vi "Main (1553).vi"() -> ()   [LabVIEW 2020]
doc: "Use this template to build a simple state machine design pattern. Each state executes code and determines which state to transition to."
uses:
  1553/_controls/1553_formatting.ctl
  1553/_controls/1553_State.ctl
  1553/_controls/1553_Data.ctl
  1553/_controls/aim1553_cluster.ctl
  1553/_controls/aim1553_messages.ctl
  1553/_controls/1553_Parameters_key.ctl
  1553/_controls/1553_Parameters.ctl
  1553/_controls/1553_minorFrames.ctl
  1553/_controls/aim1553_RT_list.ctl
  1553/_controls/ballard1553_hw_map.ctl
  1553/_controls/ballard1553_RT_list.ctl
  1553/_controls/ballard1553_cluster.ctl
  <vilib>/Utility/error.llb/DialogType.ctl
  Libraries/Aim_1553_Parameter_ni/AIM_1553_Parameter_ni.lvlib
  Libraries/Ballard_1553_Parameter_ni/Ballard_1553_Parameter_ni.lvlib
  Libraries/Ballard_1553_Hardware_ni/Ballard_1553_Hardware_ni.lvlib
  <userlib>/_OpenG.lib/array/array.llb/Sort 1D Array (DBL)__ogtk.vi
  <userlib>/_OpenG.lib/array/array.llb/Remove Duplicates from 1D Array (Variant)__ogtk.vi
  <userlib>/_OpenG.lib/array/array.llb/Search 1D Array (DBL)__ogtk.vi
  <userlib>/_OpenG.lib/array/array.llb/Index 1D Array Elements (DBL)__ogtk.vi
panel:
  out "db read time mS":u32
  in  "formatting":T1=enum."ni-AIM"
  in  "Configure SelfTestBus?":bool
  out "Progress":string
  in  "Stop Button":bool
  in  "Generate XMLs":bool
  in  "Source Filepath (xlsx)":path=path "C:/Users/Administrator/Desktop/GIT/1553-Configurator/docs/example configurations/_template_Ballard_1553.xlsx"
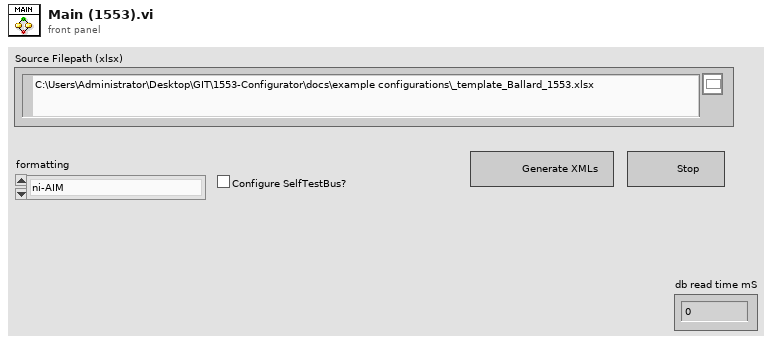
[diagram p1: front panel]
types:
  T1 = typedef "1553_formatting.ctl" = enum16{"ni-Ballard", "ni-AIM"}
  T2 = typedef "DialogType.ctl" = u16
  T3 = typedef "1553_Data.ctl" = cluster{"Database Filepath (xlsx)":path, "formatting":T1, "parameter config - aim":T4[], "hw config - aim":T9[], "hw config - ballard":T10[], "parameter config - ballard":T12[]}
  T4 = typedef "aim1553_cluster.ctl" = cluster{"messages":map{string, T5}, "parameters":map{T6, T7[]}, "frames":map{string, map{string, T8}}}
  T5 = typedef "aim1553_messages.ctl" = cluster{"messageType":string, "TA1":i32, "SA1":i32, "words":i32, "TA2":i32, "SA2":i32, "MC":i32, "direction":string}
  T6 = typedef "1553_Parameters_key.ctl" = cluster{"TA":i32, "SA":i32}
  T7 = typedef "1553_Parameters.ctl" = cluster{"name":string, "encoding":string, "signed":bool, "startBit":i32, "numberOfBits":i32, "scale":dbl, "offset":dbl, "unit":string, "defaultValue":dbl}
  T8 = typedef "1553_minorFrames.ctl" = cluster{"MessageNames":string[], "FramePeriodUs":i32}
  T9 = typedef "aim1553_RT_list.ctl" = cluster{"terminalAddress":i32[]}
  T10 = typedef "ballard1553_hw_map.ctl" = map{i32, T11}
  T11 = typedef "ballard1553_RT_list.ctl" = cluster{"terminalAddress":i32[], "channel":i32}
  T12 = typedef "ballard1553_cluster.ctl" = cluster{"messages":map{string, T5}, "parameters":map{T6, T7[]}, "frames":map{string, map{string, T8}}}
  T13 = typedef "1553_State.ctl" = enum16{"Initialize", "Wait for Event", "Read Source Files", "Validate Data", "Write Configuration Files", "Exit"}
  T14 = enum8{"Enabled", "Disabled", "Disabled and Grayed Out"}
  T15 = enum32{"invalid app kind", "Development System", "Run Time System", "Student Edition", "Embedded LabVIEW", "Evaluation", "Custom"}
  T16 = typedef "Database_Array.ctl" = cluster{"Core Number":i32, "Channel Number":i32, "Channel Name":string, "Channel Speed":i32, "Label Decimal":i32, "Label Name":string, "Min Rate (mS)":i32, "Max Rate (mS)":i32, "SDI":i32, "SSM":i32, "Create SDI":bool, "Create SSM":bool, "Create Parity":bool, "Parameter Name":string, "Start Bit":i32, "Number of Bits":i32, "Scale":string, "Offset":string, "Signed":bool, "Unit":string, "Encoding":T17, "Default Value":string}
  T17 = typedef "Encoding.ctl" = enum16{"BCD", "BNR", "Discrete"}
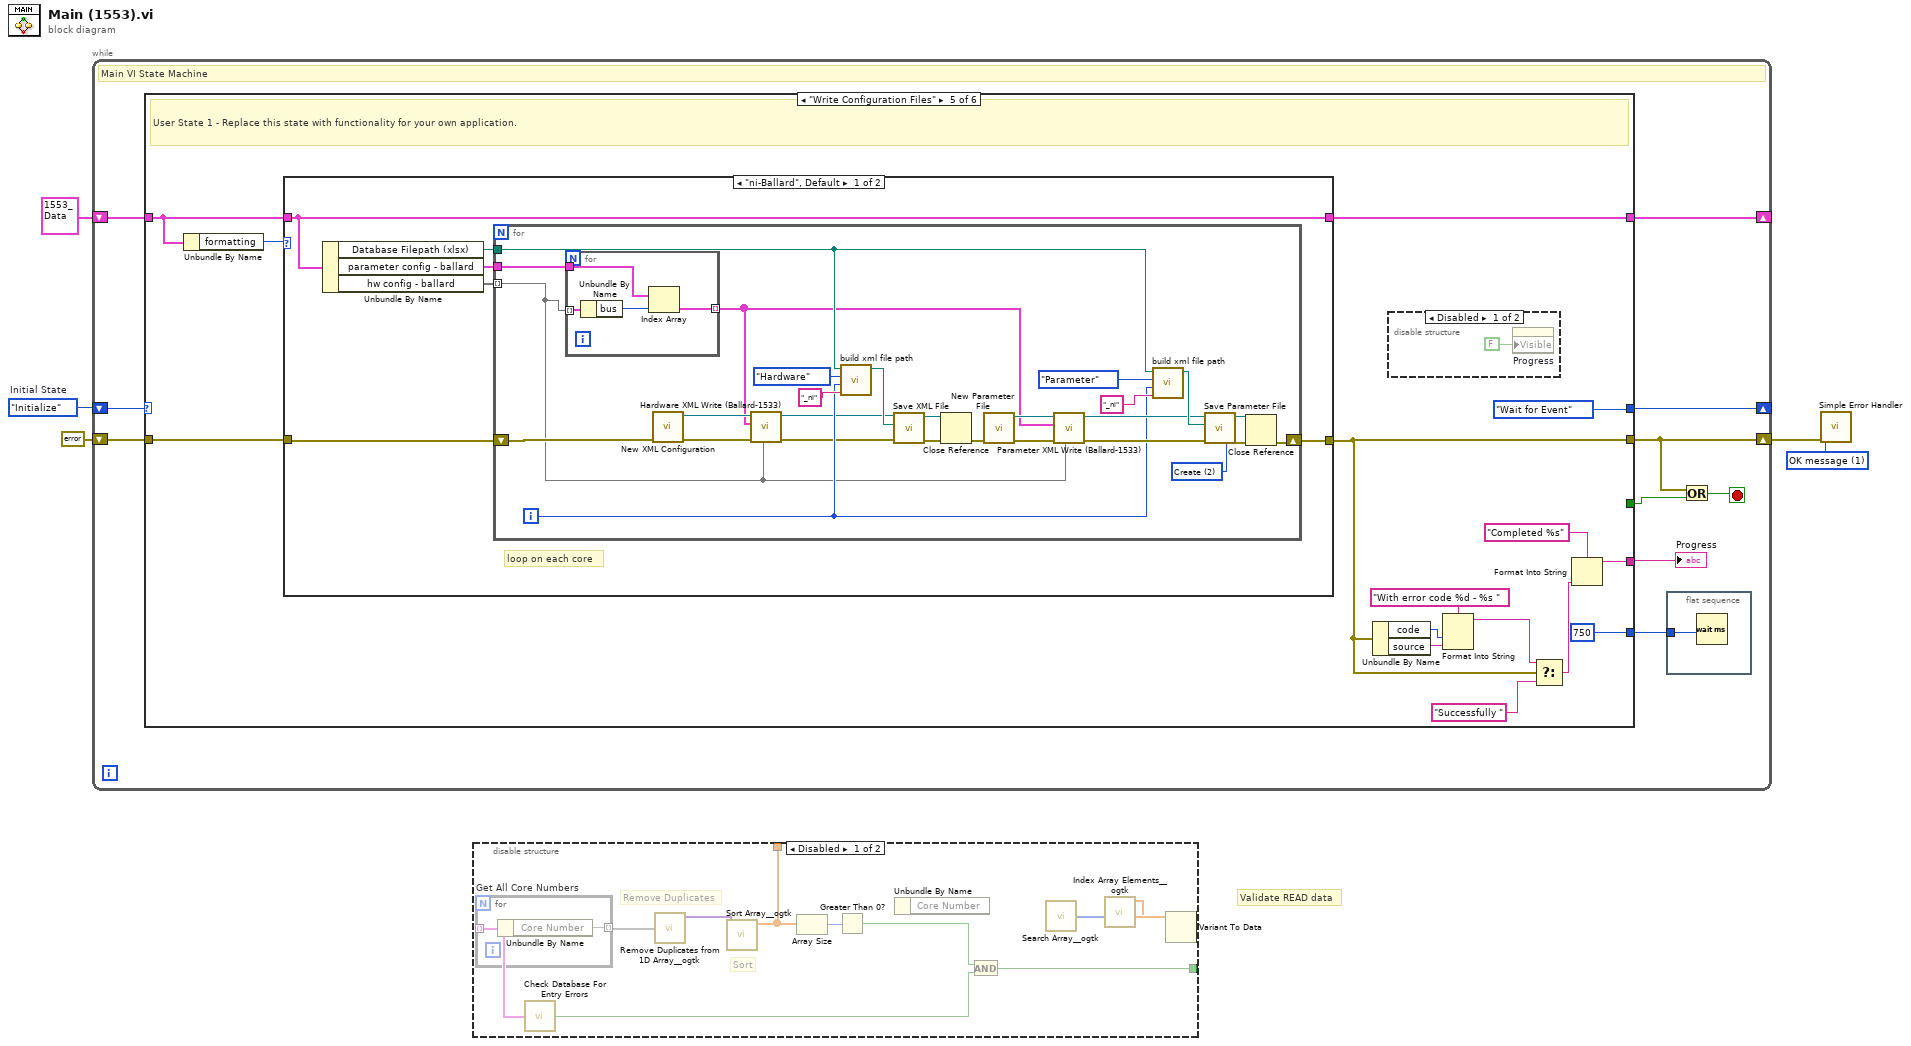
[diagram p0: block diagram]
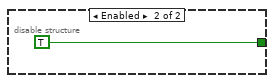
[diagram p2: hidden frame]
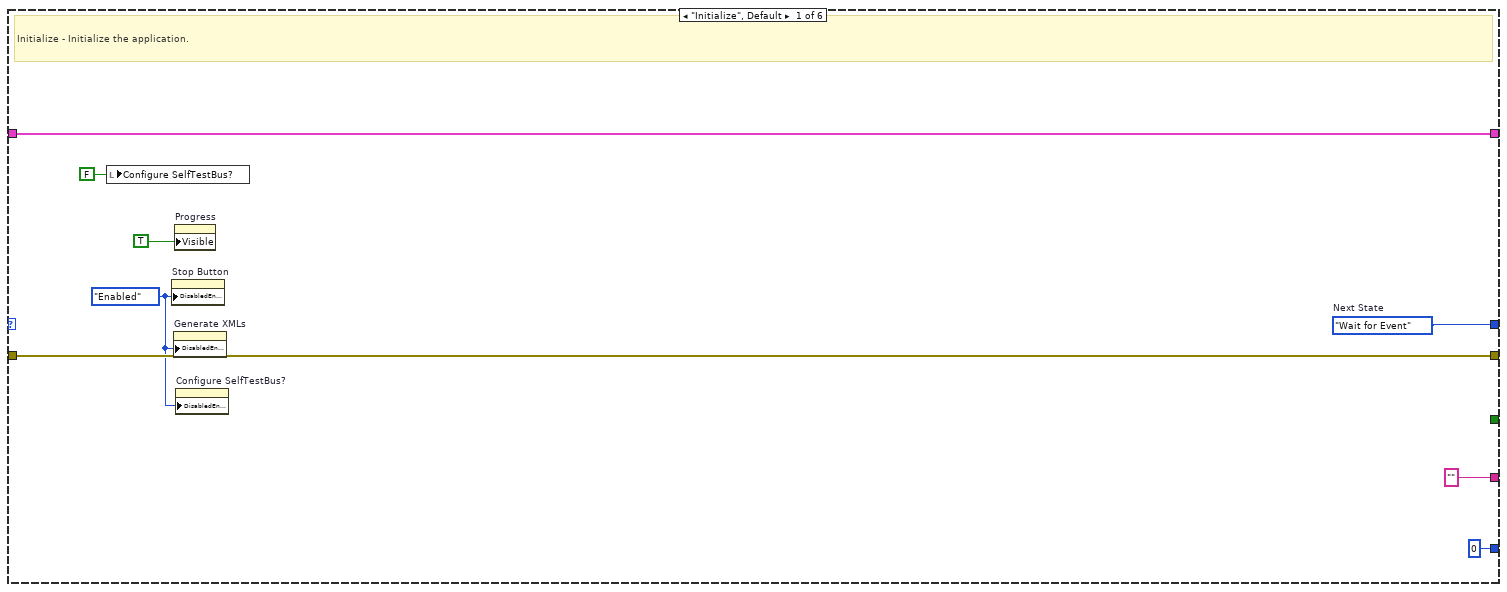
[diagram p3: hidden frame]
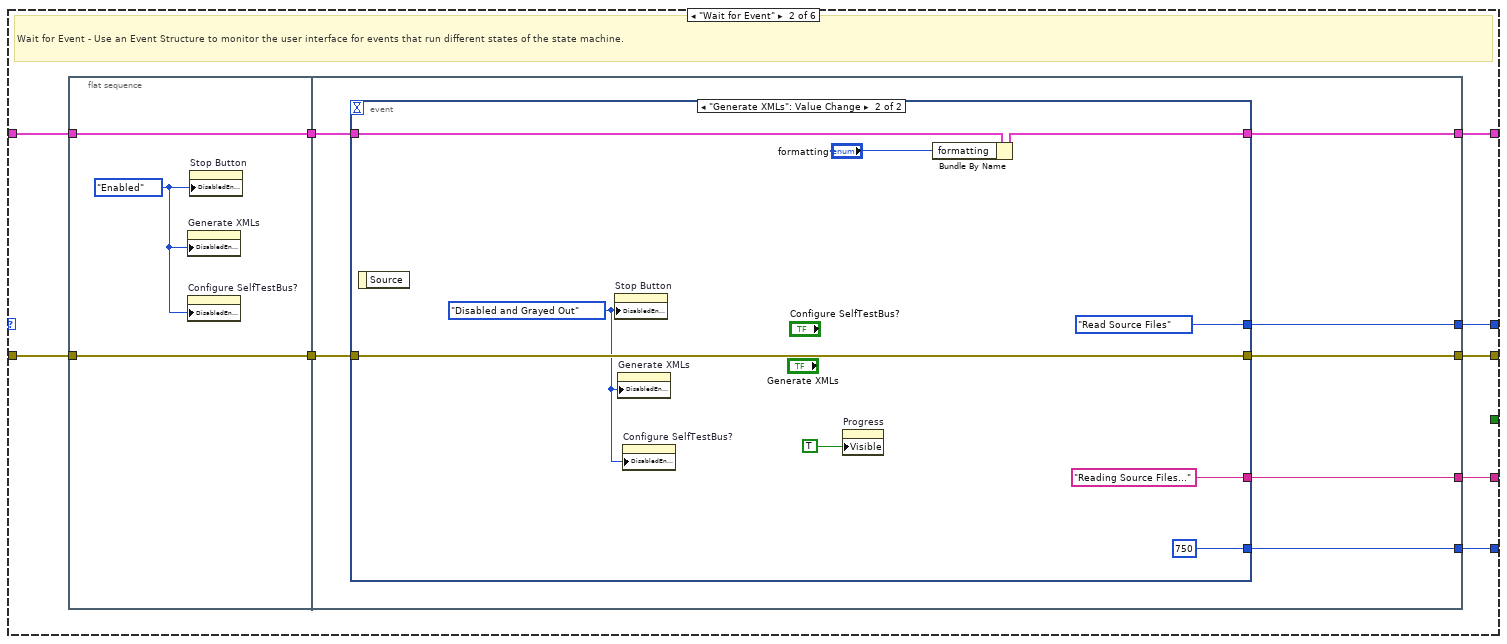
[diagram p4: hidden frame]
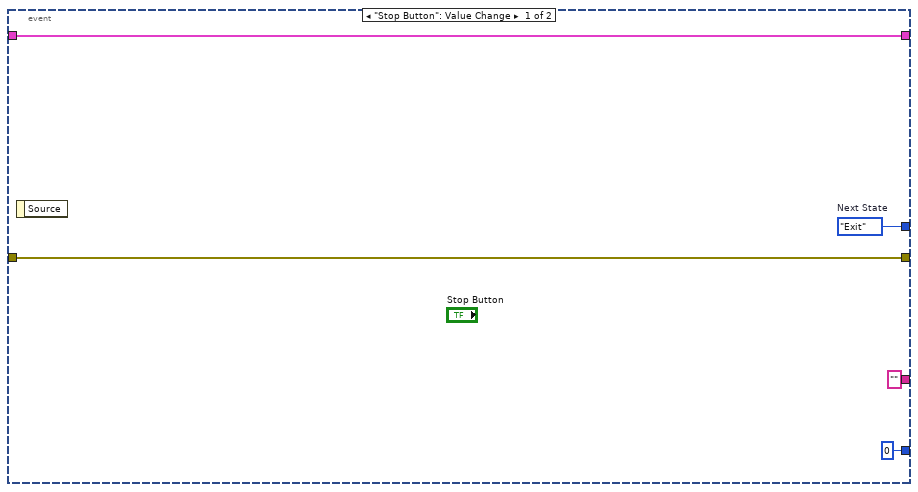
[diagram p5: hidden frame]
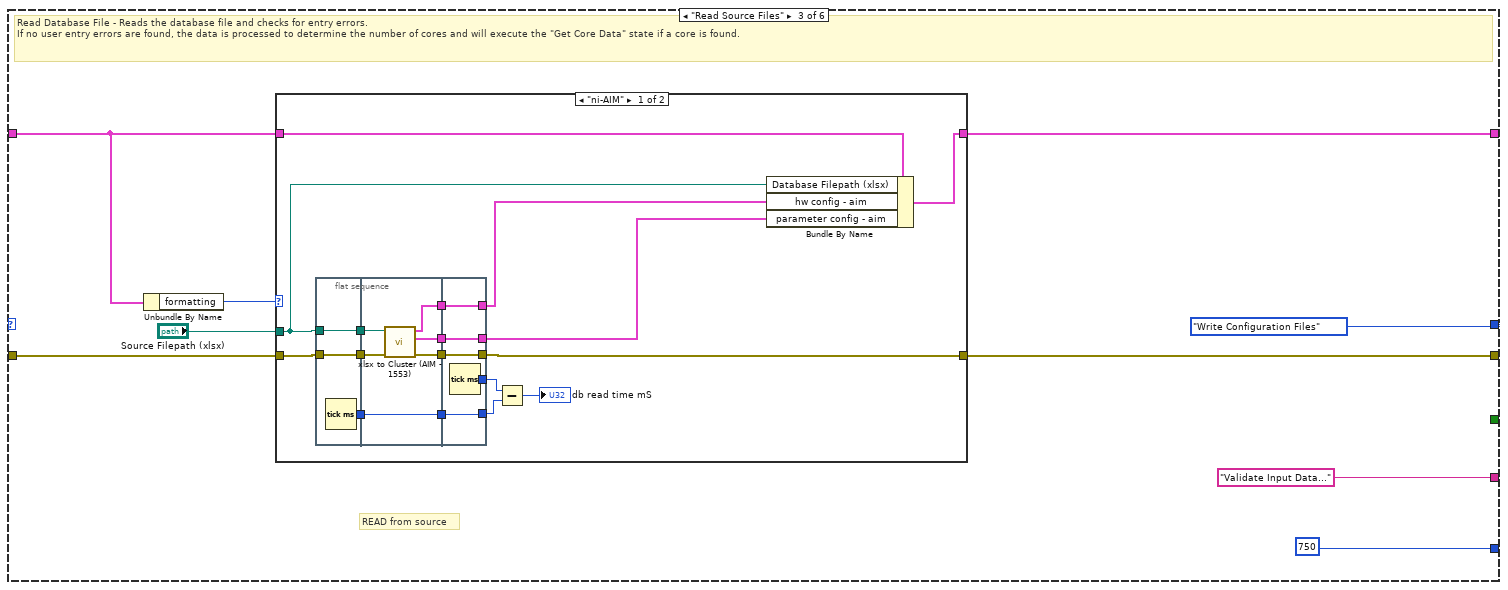
[diagram p6: hidden frame]
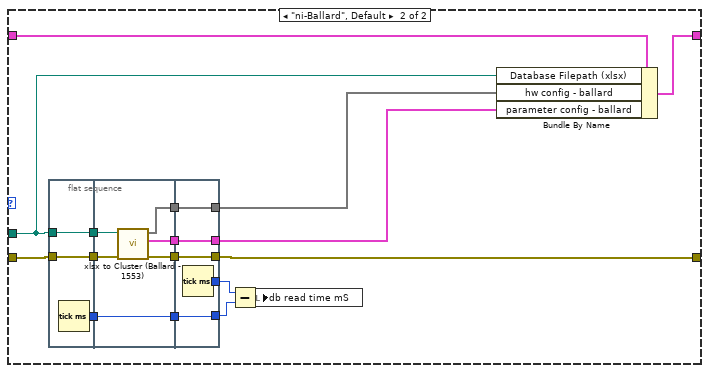
[diagram p7: hidden frame]
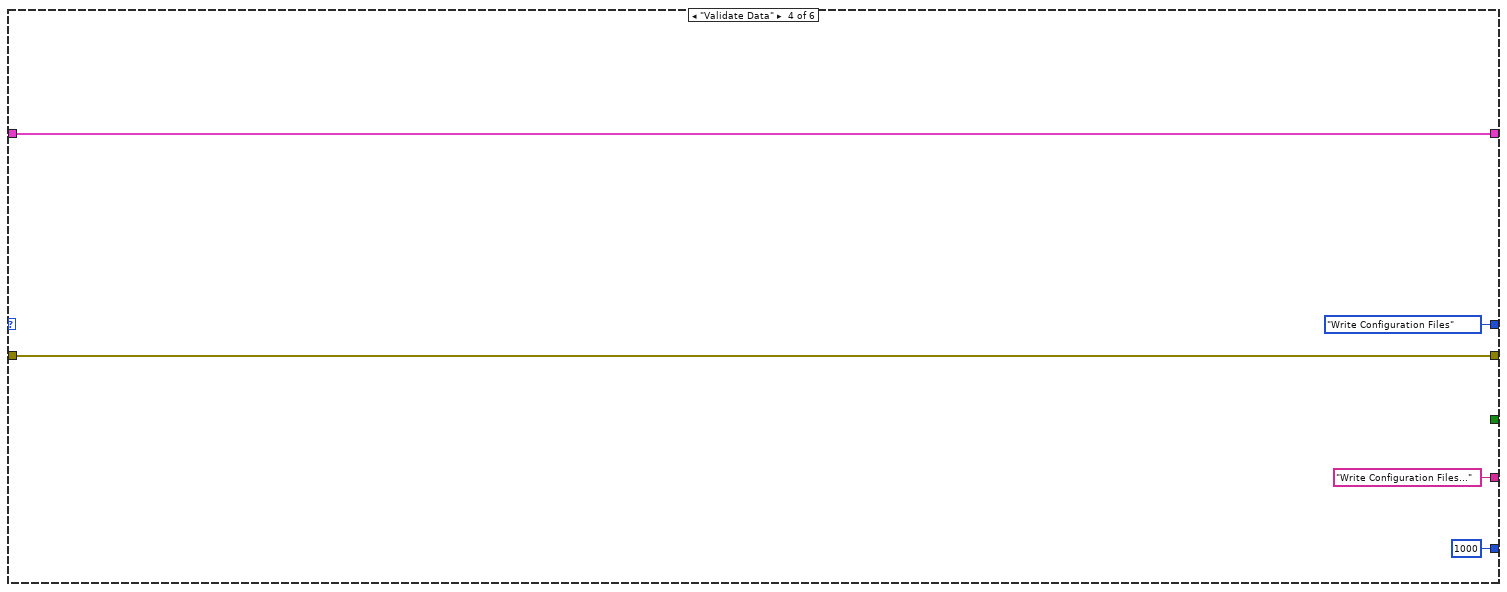
[diagram p8: hidden frame]
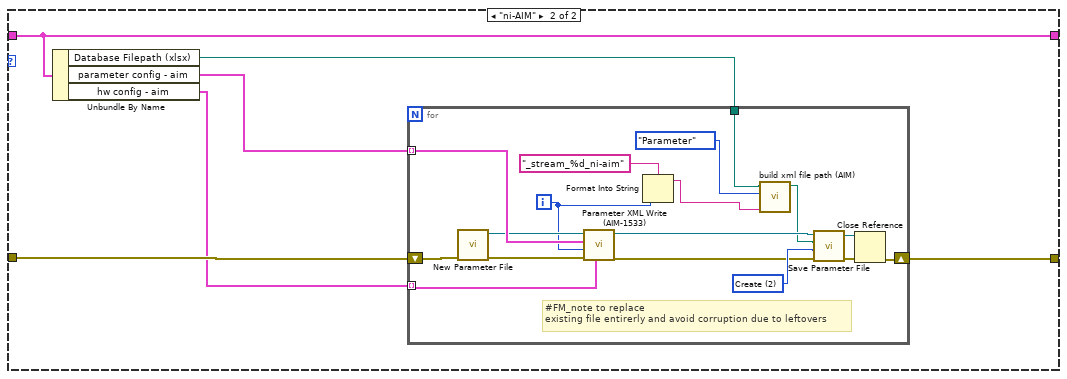
[diagram p10: hidden frame]
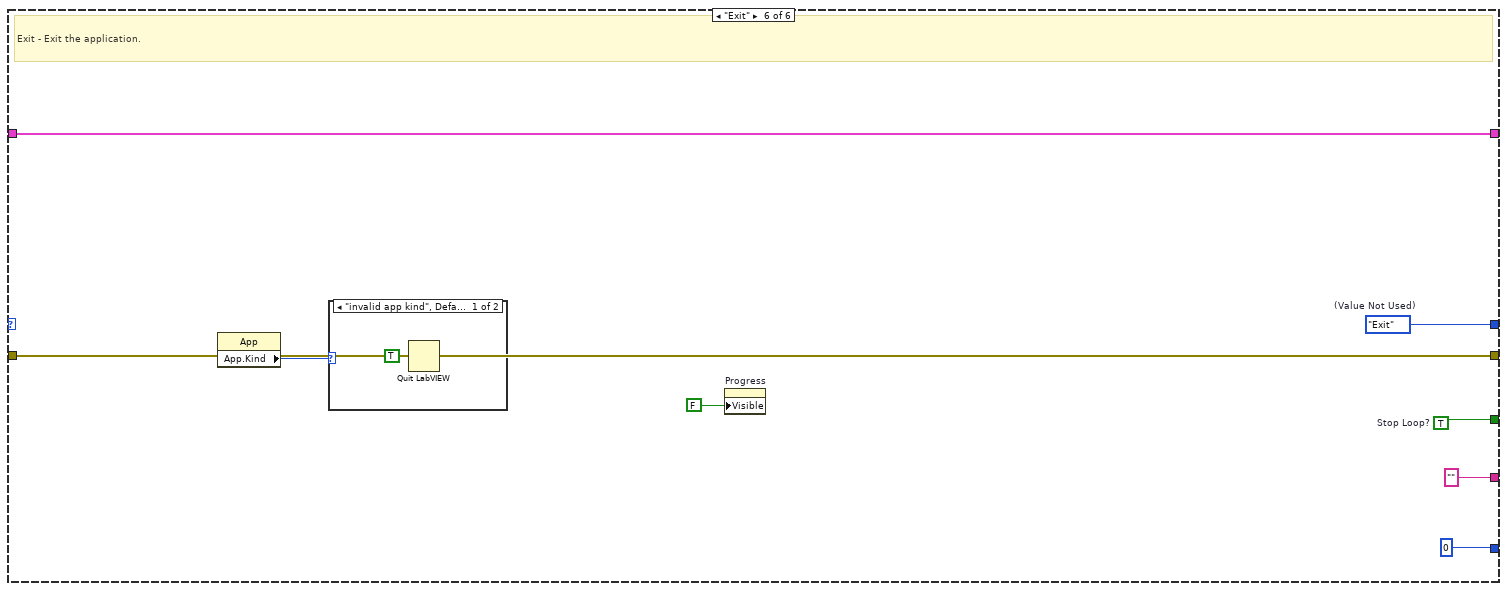
[diagram p11: hidden frame]
diagram:
  w1 = T2 1 items=["no dialog", "OK message", "continue or stop message", "OK message + warnings", "continue/stop + warnings"] ("type of dialog (OK msg:1)")
  w5 = 1553_State."Initialize"  # Initial State
  # "Validate READ data"
  n1 = while {
    shift-right: [w14] -> _
    shift-left: w5 -> [w15]
    shift-right: [w12] -> _
    shift-left: T3 {"Database Filepath (xlsx)"=path "C:/Users/jkreienh/Desktop/Preliminary Ballard Database Template.xlsx", "formatting"=enum."ni-Ballard", "parameter config - aim"=[], "hw config - aim"=[], "hw config - ballard"=[], "parameter config - ballard"=[]} ("Data") -> [w13]
    shift-right: [w7] -> w2
    shift-left: errorcluster {"status"=FALSE, "code"=0, "source"=""} ("error constant") -> [w11]
    stop <- w9 stop-if-true
    # "Main VI State Machine"
    n2 = case shown="\"Write Configuration Files\"" w15 {
      tunnel: [w24 w33 1553_State."Write Configuration Files" 1553_State."Write Configuration Files" ("(Value Not Used)") 1553_State."Wait for Event" ("Next State") w217] -> w14
      tunnel: [_ _ _ _ _ w215] -> w10
      tunnel: w13 -> [w22 w32 w61 w133 w136 w216]
      tunnel: [w22 w31 w60 w133 w134 w216] -> w12
      tunnel: w11 -> [w23 w30 w64 w132 w148 w214]
      tunnel: [w23 w29 w66 w132 w145 w214] -> w7
      tunnel: ["" w28 "Validate Input Data..." "Write Configuration Files..." w147 ""] -> w8
      tunnel: [u32 0 ("milliseconds to wait") w27 u32 750 ("milliseconds to wait") u32 1000 ("milliseconds to wait") u32 750 ("milliseconds to wait") u32 0 ("milliseconds to wait")] -> w6
      frame "Initialize", Default {
        w18 = T14."Enabled" ("Disabled")
        w24 = 1553_State."Wait for Event"  # Next State
        # "Initialize - Initialize the application."
        n3 = local write "Configure SelfTestBus?"(FALSE ("Configure SelfTestBus?")) -> ()
        n4 = property on="Stop Button" class="Bool"("DisabledEnum"=w18) -> ()  [unwired: 2 in, 2 out]
        n5 = property on="Generate XMLs" class="Bool"("DisabledEnum"=w18) -> ()  [unwired: 2 in, 2 out]
        n6 = property on="Progress" class="Str"("Visible"=TRUE) -> ()  [unwired: 2 in, 2 out]
        n7 = property on="Configure SelfTestBus?" class="Bool (strict)"("DisabledEnum"=w18) -> ()  [unwired: 2 in, 2 out]
      }
      frame "Wait for Event" {
        # "Wait for Event - Use an Event Structure to monitor the user interface for events that run different states of the state machine."
        n8 = flat-sequence {
          tunnel: w30 -> [w35]
          tunnel: w32 -> [w36]
          tunnel: [w36] -> w26
          tunnel: [w35] -> w25
          tunnel: [w43] -> w33
          tunnel: [w41] -> w31
          tunnel: [w39] -> w29
          tunnel: [w38] -> w28
          tunnel: [w37] -> w27
          tunnel: w26 -> [w42]
          tunnel: w25 -> [w40]
          frame #0 {
            w34 = T14."Enabled" ("Disabled")
            n9 = property on="Generate XMLs" class="Bool"("DisabledEnum"=w34) -> ()  [unwired: 2 in, 2 out]
            n10 = property on="Configure SelfTestBus?" class="Bool (strict)"("DisabledEnum"=w34) -> ()  [unwired: 2 in, 2 out]
            n11 = property on="Stop Button" class="Bool"("DisabledEnum"=w34) -> ()  [unwired: 2 in, 2 out]
          }
          frame #1 {
            n12 = event shown="[1] \"Generate XMLs\": Value Change" {
              selector: _ -> [_ _]
              dyn-events: _ -> [_ _]
              timeout: _ -> [_ _]
              tunnel: [w48 1553_State."Read Source Files" ("Next State")] -> w43
              tunnel: w42 -> [w47 w57]
              tunnel: [w47 w50] -> w41
              tunnel: w40 -> [w46 w56]
              tunnel: [w46 w56] -> w39
              tunnel: ["" "Reading Source Files..."] -> w38
              tunnel: [u32 0 ("milliseconds to wait") u32 750 ("milliseconds to wait")] -> w37
              event "Stop Button": Value Change {
                w48 = 1553_State."Exit"  # Next State
                n13 = event-data() -> ()  [unwired: 1 in, 1 out]
              }
              event "Generate XMLs": Value Change {
                w51 = T14."Disabled and Grayed Out" ("Disabled")
                n14 = event-data() -> ()  [unwired: 1 in, 1 out]
                n15 = property on="Stop Button" class="Bool"("DisabledEnum"=w51) -> ()  [unwired: 2 in, 2 out]
                n16 = property on="Generate XMLs" class="Bool"("DisabledEnum"=w51) -> ()  [unwired: 2 in, 2 out]
                n17 = property on="Configure SelfTestBus?" class="Bool (strict)"("DisabledEnum"=w51) -> ()  [unwired: 2 in, 2 out]
                n18 = property on="Progress" class="Str"("Visible"=TRUE) -> ()  [unwired: 2 in, 2 out]
                n19 = Bundle By Name(cluster=w57, "formatting"="formatting") -> (w50:T3)
              }
            }
          }
        }
      }
      frame "Read Source Files" {
        # "READ from source"
        # "Read Database File - Reads the database file and checks for entry errors. \nIf no user entry errors are found, the data is processed to determine the number of cores and will execute the \"Get Core Data\" state if a core is found."
        n20 = Unbundle By Name(w61) -> ("formatting"=w62:T1)
        n21 = case shown="\"ni-AIM\"" w62 {
          tunnel: [w82 w113] -> w66
          tunnel: "Source Filepath (xlsx)" -> [w69 w100]
          tunnel: w64 -> [w83 w114]
          tunnel: w61 -> [w71 w102]
          tunnel: [w70 w101] -> w60
          frame "ni-AIM" {
            n22 = flat-sequence {
              tunnel: w83 -> [w85]
              tunnel: w69 -> [w86]
              tunnel: [w86] -> w79
              tunnel: [w85] -> w78
              tunnel: [w84] -> w76
              tunnel: [w90] -> w81
              tunnel: [w89] -> w80
              tunnel: w79 -> [w92]
              tunnel: w78 -> [w91]
              tunnel: [w88] -> w77
              tunnel: w76 -> [w88]
              tunnel: [w87] -> w72
              tunnel: [w96] -> w67
              tunnel: [w97] -> w82
              tunnel: w81 -> [w97]
              tunnel: w80 -> [w96]
              tunnel: [w95] -> w75
              tunnel: [w94] -> w74
              tunnel: w77 -> [w94]
              tunnel: [w93] -> w68
              tunnel: w72 -> [w93]
              frame #0 {
                n23 = Tick Count (ms)() -> (millisecond timer value=w84:u32)
              }
              frame #1 {
                n24 = call "xlsx to Cluster (AIM - 1553).vi"("Error (in)"=w91, "file path (dialog if empty)"=w92) -> ("Error (out)"=w90:errorcluster, "Parameter Array"=w89:T4[], "hw configuration"=w87:T9[])  [unwired: 7 in]
              }
              frame #2 {
                n25 = Tick Count (ms)() -> (millisecond timer value=w95:u32)
              }
            }
            n26 = Subtract(x=w75, y=w74) -> (x-y=→"db read time mS":u32)
            n27 = Bundle By Name(cluster=w71, "Database Filepath (xlsx)"=w69, "hw config - aim"=w68, "parameter config - aim"=w67) -> (w70:T3)
          }
          frame "ni-Ballard", Default {
            n28 = flat-sequence {
              tunnel: w114 -> [w116]
              tunnel: w100 -> [w117]
              tunnel: [w117] -> w110
              tunnel: [w116] -> w109
              tunnel: [w115] -> w107
              tunnel: [w120] -> w112
              tunnel: [w119] -> w111
              tunnel: w110 -> [w121]
              tunnel: w109 -> [w122]
              tunnel: [w123] -> w108
              tunnel: w107 -> [w123]
              tunnel: [w118] -> w104
              tunnel: [w127] -> w98
              tunnel: [w128] -> w113
              tunnel: w112 -> [w128]
              tunnel: w111 -> [w127]
              tunnel: [w126] -> w106
              tunnel: [w125] -> w105
              tunnel: w108 -> [w125]
              tunnel: [w124] -> w99
              tunnel: w104 -> [w124]
              frame #0 {
                n29 = Tick Count (ms)() -> (millisecond timer value=w115:u32)
              }
              frame #1 {
                n30 = call "xlsx to Cluster (Ballard - 1553).vi"("Error (in)"=w122, "file path (dialog if empty)"=w121) -> ("Error (out)"=w120:errorcluster, "Configuration Array"=w119:T12[], "hw configuration"=w118:T10[])  [unwired: 7 in]
              }
              frame #2 {
                n31 = Tick Count (ms)() -> (millisecond timer value=w126:u32)
              }
            }
            n32 = Subtract(x=w106, y=w105) -> (x-y=w103:u32)
            n33 = local write "db read time mS"(w103) -> ()
            n34 = Bundle By Name(cluster=w102, "Database Filepath (xlsx)"=w100, "hw config - ballard"=w99, "parameter config - ballard"=w98) -> (w101:T3)
          }
        }
      }
      frame "Validate Data" {
      }
      frame "Write Configuration Files" {
        # "User State 1 - Replace this state with functionality for your own application."
        n35 = Unbundle By Name(w136) -> ("formatting"=w135:T1)
        n36 = case shown="\"ni-Ballard\", Default" w135 {
          tunnel: w148 -> [w154 w191]
          tunnel: [w155 w192] -> w145
          tunnel: w136 -> [w153 w190]
          tunnel: [w153 w190] -> w134
          frame "ni-Ballard", Default {
            # "loop on each core"
            n37 = Unbundle By Name(w153) -> ("Database Filepath (xlsx)"=w152:path, "parameter config - ballard"=w150:T12[], "hw config - ballard"=w151:T10[])
            n38 = for {
              shift-right: [w182] -> w155
              shift-left: w154 -> [w161]
              tunnel: w152 -> [w168]
              tunnel: w151 -> [w156] mode=indexing
              tunnel: w150 -> [w158]
              i -> [w169]
              w178 = 2 items=["CreateNew"=1, "Create"=2, "Open"=3, "OpenOrCreate"=4, "Truncate"=5, "Append"=6] ("mode (Create)")
              n39 = for {
                tunnel: w158 -> [w186]
                tunnel: [w185] -> w157 mode=indexing
                tunnel: w156 -> [w184] mode=indexing
                n40 = Unbundle By Name(w184) -> ("bus"=w183:i32)
                n41 = Index Array(array=w186, index=w183) -> (element=w185:T12)
              }
              n42 = call "New XML Configuration.vi"("error in"=w161) -> ("error out"=w159:errorcluster, "xml ref out"=w160:refnum<k24>)  [unwired: 9 in]
              n43 = call "Hardware XML Write (Ballard-1533).vi"("ballard_bus hw map"=w156, "error in"=w159, "configuration"=w157, "xml ref in"=w160) -> ("error out"=w162:errorcluster, "xml ref out"=w163:refnum<k24>)  [unwired: 6 in]
              n44 = call "build xml file path.vi"("additional string(\"\")"="_ni" ("additional string(\"\")"), "Core"=w169, "Filetype"=enum16{"Hardware", "Parameter"}."Hardware", "Database Filepath in"=w168) -> ("xml path out"=w164:path)  [unwired: 7 in]
              n45 = call "Save XML File.vi"("error in"=w162, "XML Configuration File Path"=w164, "xml ref in"=w163) -> ("error out"=w167:errorcluster, "xml ref out"=w165:refnum<k24>)  [unwired: 7 in]
              n46 = Close Reference(reference=w165, error in (no error)=w167) -> (error out=w166:errorcluster)
              n47 = call "New Parameter File.vi"("error in"=w166) -> ("error out"=w173:errorcluster, "new parameter file"=w174:refnum<k24>)  [unwired: 9 in]
              n48 = call "Parameter XML Write (Ballard-1533).vi"("ballard_bus hw map"=w156, "error in"=w173, "configuration"=w157, "parameter file in"=w174) -> ("error out"=w172:errorcluster, "parameter file out"=w175:refnum<k24>)  [unwired: 6 in]
              n49 = call "build xml file path.vi"("additional string(\"\")"="_ni" ("additional string(\"\")"), "Core"=w169, "Filetype"=enum16{"Hardware", "Parameter"}."Parameter", "Database Filepath in"=w168) -> ("xml path out"=w179:path)  [unwired: 7 in]
              n50 = call "Save Parameter File.vi"("error in"=w172, "mode (Create)"=w178, "XML path"=w179, "parameter file in"=w175) -> ("error out"=w177:errorcluster, "parameter file out"=w176:refnum<k24>)  [unwired: 5 in, 1 out]
              n51 = Close Reference(reference=w176, error in (no error)=w177) -> (error out=w182:errorcluster)
            }
          }
          frame "ni-AIM" {
            n52 = Unbundle By Name(w190) -> ("Database Filepath (xlsx)"=w189:path, "parameter config - aim"=w188:T4[], "hw config - aim"=w187:T9[])
            n53 = for {
              tunnel: w188 -> [w208] mode=indexing
              tunnel: w187 -> [w199] mode=indexing
              tunnel: w189 -> [w198]
              shift-right: [w209] -> w192
              shift-left: w191 -> [w207]
              i -> [w193]
              w204 = 2 items=["CreateNew"=1, "Create"=2, "Open"=3, "OpenOrCreate"=4, "Truncate"=5, "Append"=6] ("mode (Create)")
              # "#FM_note to replace \nexisting file entirerly and avoid corruption due to leftovers"
              n54 = call "New Parameter File.vi"("error in"=w207) -> ("error out"=w201:errorcluster, "new parameter file"=w200:refnum<k24>)  [unwired: 9 in]
              n55 = call "Parameter XML Write (AIM-1533).vi"("hw configuration"=w199, "error in"=w201, "hardwareChannel"=w193, "aim1553_cluster"=w208, "parameter file in"=w200) -> ("error out"=w203:errorcluster, "parameter file out"=w202:refnum<k24>)  [unwired: 5 in]
              n56 = Format Into String(format string="_stream_%d_ni-aim" ("additional string(\"\")"), w193) -> (resulting string=w195:string)  [unwired: 2 in, 1 out]
              n57 = call "build xml file path (AIM).vi"("additional string(\"\")"=w195, "Filetype"=enum16{"Hardware", "Parameter"}."Parameter", "Database Filepath in"=w198) -> ("xml path out"=w196:path)  [unwired: 8 in]
              n58 = call "Save Parameter File.vi"("error in"=w203, "mode (Create)"=w204, "XML path"=w196, "parameter file in"=w202) -> ("error out"=w206:errorcluster, "parameter file out"=w205:refnum<k24>)  [unwired: 5 in, 1 out]
              n59 = Close Reference(reference=w205, error in (no error)=w206) -> (error out=w209:errorcluster)
            }
          }
        }
        n60 = Unbundle By Name(w145) -> ("code"=w142:i32, "source"=w141:string)
        n61 = disable-structure shown="Disabled" {
          frame Disabled {
            n62 = property on="Progress" class="Str"("Visible"=FALSE) -> ()  [unwired: 2 in, 2 out]
          }
          frame Enabled {
          }
        }
        n63 = Format Into String(format string="With error code %d - %s ", w142, w141) -> (resulting string=w139:string)  [unwired: 2 in, 1 out]
        n64 = Select(t=w139, s=w145, f="Successfully ") -> (s? t:f=w140:string)
        n65 = Format Into String(format string="Completed %s", w140) -> (resulting string=w147:string)  [unwired: 2 in, 1 out]
      }
      frame "Exit" {
        w215 = TRUE  # Stop Loop?
        w217 = 1553_State."Exit"  # (Value Not Used)
        # "Exit - Exit the application."
        n66 = property class="App"() -> ("App.Kind"=w210:T15)  [unwired: 2 in, 2 out]
        n67 = case shown="\"invalid app kind\", Default" w210 {
          frame "invalid app kind", Default {
            n68 = Quit LabVIEW(quit? (T)=TRUE) -> ()
          }
          frame "Development System" {
          }
        }
        n69 = property on="Progress" class="Str"("Visible"=FALSE) -> ()  [unwired: 2 in, 2 out]
      }
    }
    "Progress" <- w8
    n70 = flat-sequence {
      tunnel: w6 -> [w16]
      frame #0 {
        n71 = Wait (ms)(milliseconds to wait=w16) -> ()  [unwired: 1 out]
      }
    }
    n72 = Or(x=w7, y=w10) -> (x .or. y?=w9:bool)
  }
  n73 = disable-structure shown="Disabled" {
    disable-tunnel: [w227 _] -> _
    disable-tunnel: [w224 TRUE] -> _
    frame Disabled {
      # "Sort"
      # "Remove Duplicates"
      n74 = call "Check Database For Entry Errors.vi"() -> ("All Parameters Array"=w228:T16[], "Database OK?"=w225:bool)  [unwired: 14 in]
      n75 = for "Get All Core Numbers" {
        tunnel: w228 -> [w233] mode=indexing
        tunnel: [w232] -> w231 mode=indexing
        n76 = Unbundle By Name(w233) -> ("Core Number"=w232)
      }
      n77 = call-poly <userlib>:"Remove Duplicates from 1D Array__ogtk.vi"("Input Array"=w231) -> ("Output Array"=w230:variant[])  [unwired: 1 out]
      n78 = call-poly <userlib>:"Sort Array__ogtk.vi"("Array in"=w230) -> ("Sorted Array out"=w227:dbl[])  [unwired: 9 in, 1 out]
      n79 = Array Size(array=w227) -> (size(s)=w229:i32)
      n80 = Greater Than 0?(x=w229) -> (x > 0?=w226:bool)
      n81 = Unbundle By Name() -> ("Core Number"=w223:i32)  [unwired: 1 in]
      n82 = And(x=w226, y=w225) -> (x .and. y?=w224:bool)
      n83 = call-poly <userlib>:"Search Array__ogtk.vi"() -> ("Array"=w219:dbl[], "Indices of Elements"=w220:i32[])  [unwired: 8 in]
      n84 = call-poly <userlib>:"Index Array Elements__ogtk.vi"("indices"=w220) -> ("elements"=w222:dbl[], "array"=w221:dbl[])  [unwired: 9 in]
      n85 = Variant To Data(type=w221, Variant=w222) -> ()  [unwired: 1 in, 2 out]
    }
    frame Enabled {
    }
  }
  n86 = call <vilib>:"Simple Error Handler.vi"("type of dialog (OK msg:1)"=w1, "error in (no error)"=w2) -> ()  [unwired: 3 in, 5 out]
